vi "Destroy_Stop_Event.vi"(8 "error in (no error)":errorcluster={"status"=FALSE, "code"=0, "source"="\"\""}, 11 "User Event - Stop":refnum<user-event>) -> (0 "error out":errorcluster)   [LabVIEW 2026]
doc: "Destroy the user event."
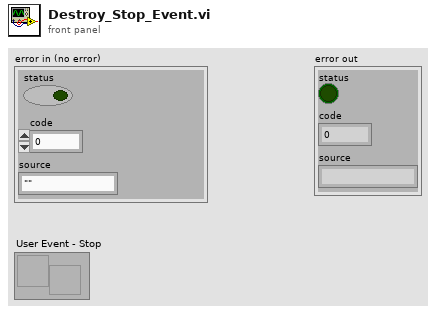
[diagram p1: front panel]
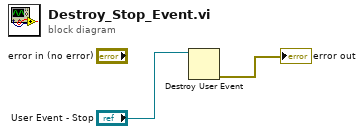
[diagram p0: block diagram]
diagram:
  n1 = Destroy User Event(user event="User Event - Stop") -> (error out=→"error out":errorcluster)  [unwired: 1 in]
